vi "Variant to String.vi"(8 "error in (no error)":errorcluster, 10 "Variant":variant, 11 "StringFormatter in":refnum<class "StringFormatter.lvclass">) -> (0 "error out":errorcluster, 2 "Value":string, 3 "StringFormatter out":refnum<class "StringFormatter.lvclass">)   [LabVIEW 2013, in "OpenStringFormatter.lvlib" / "StringFormatter.lvclass"]
uses:
  StringFormatter.lvclass
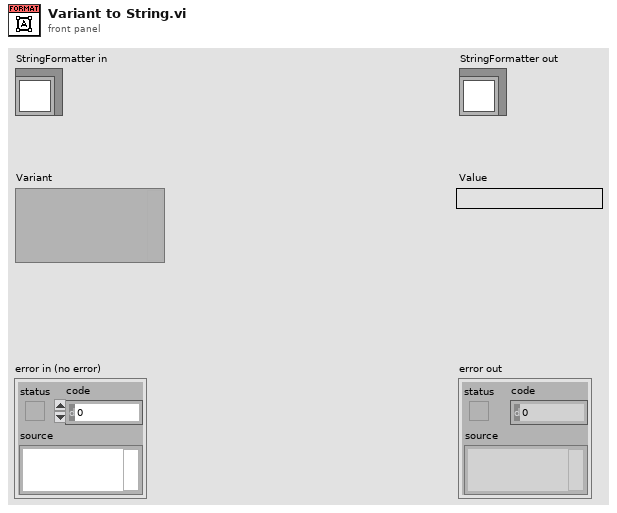
[diagram p1: front panel]
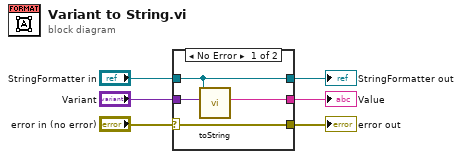
[diagram p0: block diagram]
diagram:
  n1 = case shown="No Error" "error in (no error)" {
    selector: "error in (no error)" -> [w7 w12]
    tunnel: [w7 w12] -> w5
    tunnel: [w8 w11] -> w3
    tunnel: "StringFormatter in" -> [w8 w11]
    tunnel: "Variant" -> [w10 _]
    tunnel: [w9 _] -> w1
    frame No Error {
      n2 = call-dynamic "toString.vi"("Variant"=w10, "StringFormatter in"=w8) -> ("Value"=w9:string)  [unwired: 9 in]
    }
    frame Error {
    }
  }
  "error out" <- w5
  "StringFormatter out" <- w3
  "Value" <- w1
